vi "Process.vi"(8 "error in":errorcluster, 11 "Qbus in":refnum<class "Qbus.lvclass">) -> (0 "error out":errorcluster)   [LabVIEW 2021, in "AudioGenTCPReaderProcess.lvlib"]
uses:
  AudioGenTCPReaderProcess.lvlib
  <vilib>/addons/Qbus/Qbus.lvclass
  <vilib>/NI/STM/TCP/TCP Read Options.ctl
  shared/logger process/controls/event.ctl
  controls/digital generation settings.ctl
  controls/digital protocol settings.ctl
  <vilib>/PDM Acquisition Toolkit/host/Classes/Session/Controls/Logic Levels.ctl
  <vilib>/PDM Acquisition Toolkit/shared/controls/PCM Data Format Configuration.ctl
  <vilib>/PDM Acquisition Toolkit/shared/controls/Digital Edge.ctl
  <vilib>/PDM Acquisition Toolkit/shared/controls/PCM Bit Endianness.ctl
  <vilib>/PDM Acquisition Toolkit/shared/controls/PCM Data Justification.ctl
  <vilib>/PDM Acquisition Toolkit/shared/controls/clock mode.ctl
  <vilib>/PDM Acquisition Toolkit/shared/controls/PCM Frame Sync Control.ctl
  controls/signal settings.ctl
  controls/signal type.ctl
  shared/controls/digital output level units.ctl
  controls/analog generation settings.ctl
  controls/analog output settings.ctl
  controls/terminal configuration.ctl
  <vilib>/NI/STM/TCP/Read Message (TCP).vi
  <vilib>/NI/STM/TCP/Write Message (TCP).vi
  ManageConnection/AudioGenManageConnectionProcess.lvlib
  <vilib>/NI/STM/NI STM.lvlib
  shared/logger process/EventLoggerProcess.lvlib
  Digital Audio Generation/DigitalAudioGenerationProcess.lvlib
  <vilib>/PDM Acquisition Toolkit/host/Classes/Session/DecoderSession.lvclass
  <vilib>/PDM Acquisition Toolkit/shared/PDM Shared.lvlib
  controls/AudioGenTypeDefs.lvlib
  subVIs/utility/AudioGenUtility.lvlib
  Analog Generation/AnalogGenerationProcess.lvlib
  shared/controls/audio controls.lvlib
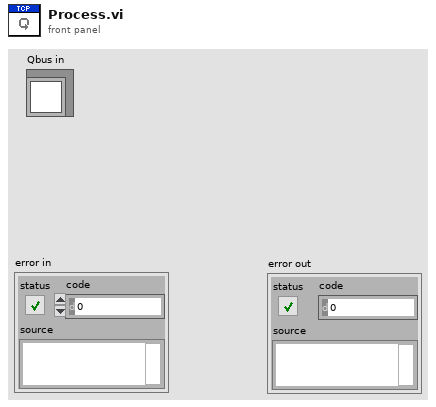
[diagram p1: front panel]
types:
  T1 = typedef "NI STM.lvlib/TCP Read Options.ctl" = cluster{"ignore timeout error":bool, "timeout ms (1000)":i32}
  T2 = typedef "EventLoggerProcess.lvlib/event.ctl" = cluster{"name":string, "description":string}
  T3 = typedef "AudioGenTypeDefs.lvlib/digital generation settings.ctl" = cluster{"data channel list":string, "master clock channel list":string, "digital protocol settings":T4, "signal settings":T12}
  T4 = typedef "AudioGenTypeDefs.lvlib/digital protocol settings.ctl" = cluster{"logic level":T5, "PCM Data Configuration":T6, "bit clock rate":sgl, "master clock rate":sgl, "clock mode":T10, "Frame Sync Clock Control":T11}
  T5 = typedef "PDM Acquisition Class Library.lvlib/DecoderSession.lvclass/Logic Levels.ctl" = enum16{"3.3 V", "1.8 V", "1.2 V"}
  T6 = typedef "PDM Shared.lvlib/PCM Data Format Configuration.ctl" = cluster{"Frame Sync Edge for Channel 0":T7, "Channel Count Per Frame":u8, "Channel Length":u16, "Bit Depth":u8, "Channel 0 Offset":u16, "Endianness":T8, "Data Justification":T9}
  T7 = typedef "PDM Shared.lvlib/Digital Edge.ctl" = enum8{"Rising", "Falling"}
  T8 = typedef "PDM Shared.lvlib/PCM Bit Endianness.ctl" = enum16{"MSB First", "LSB First"}
  T9 = typedef "PDM Shared.lvlib/PCM Data Justification.ctl" = enum16{"Left Justified", "Right Justified"}
  T10 = typedef "PDM Shared.lvlib/clock mode.ctl" = enum16{"divided clock", "DDS"}
  T11 = typedef "PDM Shared.lvlib/PCM Frame Sync Control.ctl" = cluster{"Frame Length":u16, "Frame Sync Pulse Width":u16, "Bit Clock Edge  Sync":T7}
  T12 = typedef "AudioGenTypeDefs.lvlib/signal settings.ctl" = cluster{"signal type":T13, "properties":string, "output level units":T14}
  T13 = typedef "AudioGenTypeDefs.lvlib/signal type.ctl" = enum16{"Sine", "Dual Tone"}
  T14 = typedef "audio controls.lvlib/digital output level units.ctl" = enum32{"% FS", "dBFS", "V"}
  T15 = typedef "AudioGenTypeDefs.lvlib/analog generation settings.ctl" = cluster{"channel list":string, "output settings":T16, "signal settings":T12}
  T16 = typedef "AudioGenTypeDefs.lvlib/analog output settings.ctl" = cluster{"output rate":dbl, "range":dbl, "terminal configuration":T17, "output impedance":dbl, "common mode offset":dbl, "pure tone mode":bool}
  T17 = typedef "AudioGenTypeDefs.lvlib/terminal configuration.ctl" = enum32{"Default", "RSE", "Differential", "Pseudodifferential"}
  T18 = typedef "AudioGenTypeDefs.lvlib/service settings.ctl" = cluster{"port":u32, "enable debug log":bool}
  T19 = typedef "NI STM.lvlib/TCP Connection Info.ctl" = cluster{"connection ID":refnum<k5>, "meta data":T20[]}
  T20 = typedef "NI STM.lvlib/MetaDataElement.ctl" = string
  T21 = typedef "AudioGenTypeDefs.lvlib/generation type and status.ctl" = cluster{"status":T22, "generation type":T23}
  T22 = typedef "AudioGenTypeDefs.lvlib/generation status.ctl" = enum16{"Idle", "Committed", "Active"}
  T23 = typedef "AudioGenTypeDefs.lvlib/generation type.ctl" = enum16{"analog", "digital"}
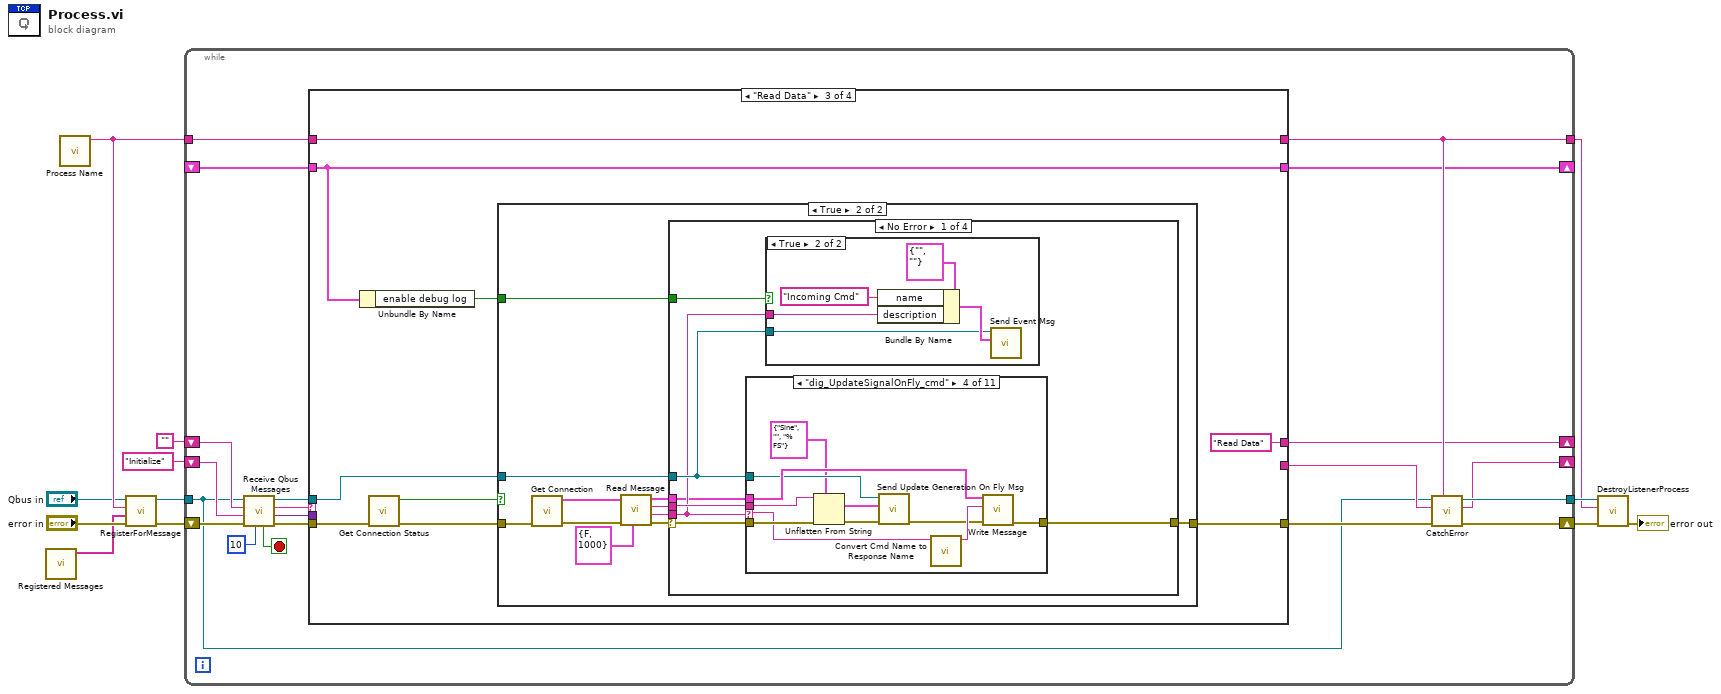
[diagram p0: block diagram]
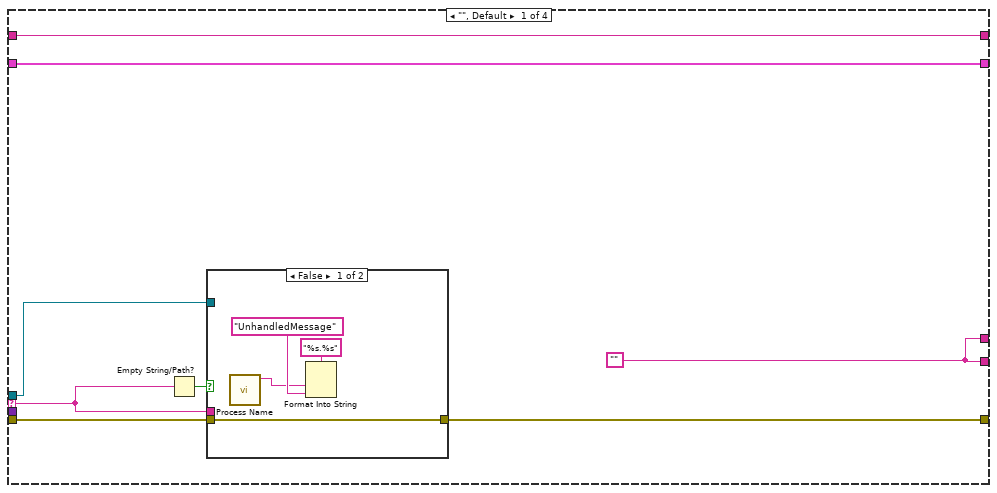
[diagram p2: hidden frame]
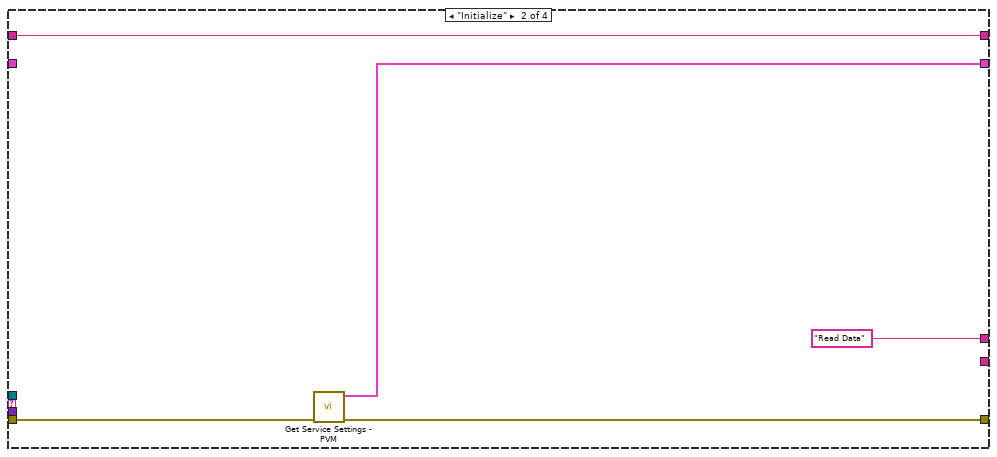
[diagram p4: hidden frame]
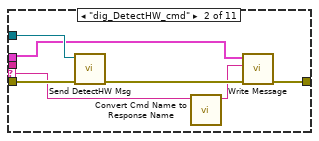
[diagram p8: hidden frame]
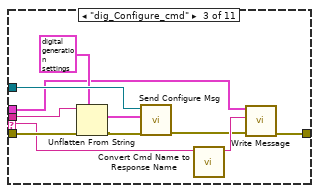
[diagram p9: hidden frame]
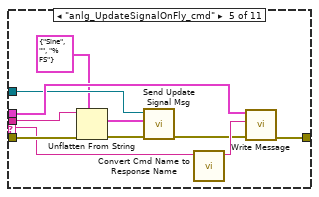
[diagram p10: hidden frame]
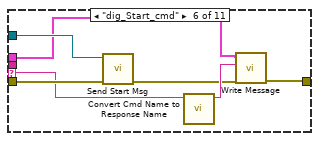
[diagram p11: hidden frame]
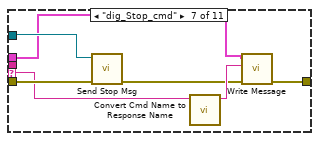
[diagram p12: hidden frame]
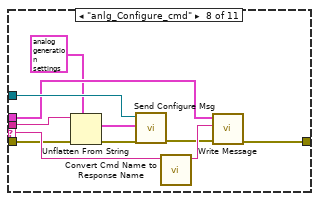
[diagram p13: hidden frame]
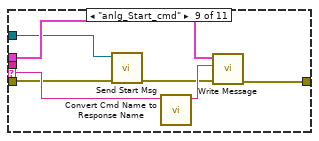
[diagram p14: hidden frame]
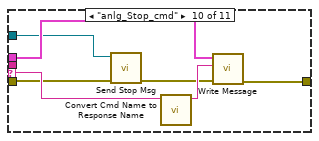
[diagram p15: hidden frame]
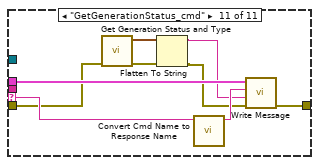
[diagram p16: hidden frame]
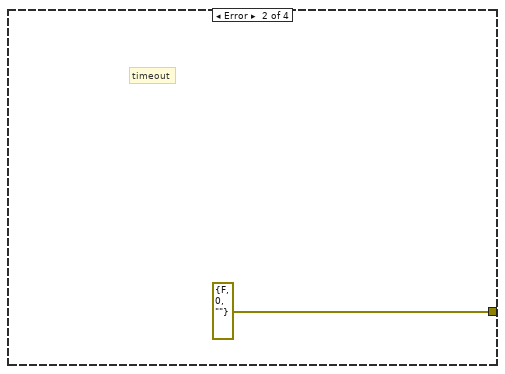
[diagram p17: hidden frame]
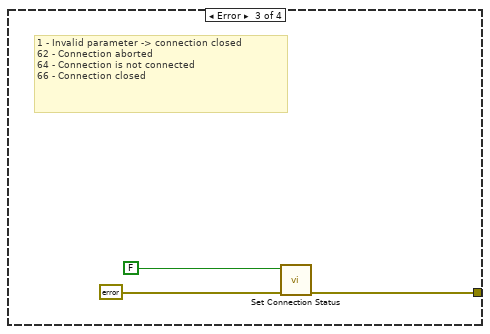
[diagram p18: hidden frame]
diagram:
  n1 = call "Registered Messages.vi"() -> ("registered messages"=w5:string[])  [unwired: 11 in]
  n2 = call "Process Name.vi"() -> ("process name"=w8:string)  [unwired: 11 in]
  n3 = call <vilib>:"RegisterForMessage.vi"("error in (no error)"="error in", "message names"=w5, "process name"=w8, "Qbus in"="Qbus in") -> ("error in (no error)"=w11:errorcluster, "Qbus out"=w12:refnum<class "Qbus.lvclass">)  [unwired: 6 in]
  n4 = while {
    shift-right: [w18] -> _
    shift-left: "" -> [w31]
    tunnel: w12 -> [w16]
    tunnel: w8 -> [w15]
    tunnel: [w25] -> w3
    tunnel: [w20] -> w1
    shift-right: [w24] -> _
    shift-left: "Initialize" -> [w27]
    shift-right: [w26] -> w4
    shift-left: w11 -> [w23]
    shift-right: [w14] -> _
    shift-left: _ -> [w13]
    stop <- w32 stop-if-true
    n5 = call "Receive Qbus Messages.vi"("timeout(ms)"=10 ("milliseconds to wait"), "error in (no error)"=w23, "priority action"=w27, "default action"=w31, "Qbus in"=w16) -> ("error out"=w30:errorcluster, "message value"=w28:variant, "action"=w22:string, "Qbus out"=w29:refnum<class "Qbus.lvclass">, "exit"=w32:bool)  [unwired: 2 in]
    n6 = case shown="\"Read Data\"" w22 {
      selector: w22 -> [w37 _ _ _]
      tunnel: w30 -> [w39 w48 w58 w180]
      tunnel: w29 -> [w35 _ w54 _]
      tunnel: [w38 w47 w53 w180] -> w17
      tunnel: w28 -> [_ _ _ _]
      tunnel: [w40 w50 w59 w179] -> w20
      tunnel: w15 -> [w40 w50 w59 w179]
      tunnel: [w34 _ _ _] -> w19
      tunnel: [w34 "Read Data" "Read Data" _] -> w18
      tunnel: [w33 w46 w52 w178] -> w14
      tunnel: w13 -> [w33 _ w52 w178]
      frame "", Default {
        w34 = ""
        n7 = Empty String/Path?(string/path=w37) -> (empty?=w36:bool)
        n8 = case shown="False" w36 {
          tunnel: [w41 w45] -> w38
          tunnel: w39 -> [w41 w45]
          tunnel: w37 -> [_ _]
          tunnel: w35 -> [_ _]
          frame False {
            n9 = call "Process Name.vi"() -> ("process name"=w42:string)  [unwired: 11 in]
            n10 = Format Into String(format string="%s.%s", w42, "UnhandledMessage" ("ProcessName")) -> ()  [unwired: 2 in, 2 out]
          }
          frame True {
          }
        }
      }
      frame "Initialize" {
        n11 = call "Get Service Settings - PVM.vi"("error in (no error)"=w48) -> ("error out"=w47:errorcluster, "service settings"=w46:T18)  [unwired: 9 in]
      }
      frame "Read Data" {
        n12 = Unbundle By Name(w52) -> ("enable debug log"=w51:bool)
        n13 = call "Get Connection Status.vi"("error in (no error)"=w58) -> ("error out"=w56:errorcluster, "connected"=w57:bool)  [unwired: 9 in]
        n14 = case shown="True" w57 {
          tunnel: w56 -> [w60 w71]
          tunnel: [w60 w65] -> w53
          tunnel: w54 -> [_ w68]
          tunnel: w51 -> [_ w61]
          frame False {
          }
          frame True {
            n15 = call "Get Connection.vi"("error in (no error)"=w71) -> ("error out"=w70:errorcluster, "connection"=w69:T19)  [unwired: 9 in]
            n16 = call-poly <vilib>:"Read Message.vi"("options"=T1 {"ignore timeout error"=FALSE, "timeout ms (1000)"=1000}, "error in"=w70, "connection info in"=w69) -> ("error out"=w63:errorcluster, "name"=w66:T20, "data string"=w67:string, "connection info out"=w62:T19)  [unwired: 3 in, 2 out]
            n17 = case shown="No Error" w63 {
              selector: w63 -> [w77 _ _ w177]
              tunnel: w68 -> [w78 _ _ _]
              tunnel: w67 -> [w76 _ _ _]
              tunnel: w66 -> [w75 _ _ _]
              tunnel: [w73 errorcluster {"status"=FALSE, "code"=0, "source"=""} ("error out") w176 w177] -> w65
              tunnel: w62 -> [w74 _ _ _]
              tunnel: w61 -> [w72 _ _ _]
              frame No Error {
                n18 = case shown="\"dig_UpdateSignalOnFly_cmd\"" w75 {
                  selector: w75 -> [_ w86 w93 w109 w120 w125 w132 w145 w154 w161 w169]
                  tunnel: w77 -> [w84 w91 w101 w113 w124 w131 w137 w143 w151 w159 w166]
                  tunnel: [w84 w88 w92 w108 w119 w127 w134 w147 w155 w162 w170] -> w73
                  tunnel: w78 -> [_ w90 w102 w105 w116 w130 w138 w146 w152 w157 _]
                  tunnel: w76 -> [_ _ w99 w112 w123 _ _ w141 _ _ _]
                  tunnel: w74 -> [_ w87 w94 w110 w121 w126 w133 w144 w153 w160 w171]
                  frame "", Default {
                  }
                  frame "dig_DetectHW_cmd" {
                    n19 = call "Send DetectHW Msg.vi"("error in"=w91, "Qbus in"=w90) -> ("error out"=w89:errorcluster)  [unwired: 8 in, 1 out]
                    n20 = call "Convert Cmd Name to Response Name.vi"("cmd name"=w86) -> ("response name"=w85:string)  [unwired: 10 in]
                    n21 = call-poly <vilib>:"Write Message.vi"("error in"=w89, "name"=w85, "connection info in"=w87) -> ("error out"=w88:errorcluster)  [unwired: 7 in, 1 out]
                  }
                  frame "dig_Configure_cmd" {
                    n22 = Unflatten From String(type=T3 {"data channel list"="", "master clock channel list"="", "digital protocol settings"={"logic level"=enum."3.3 V", "PCM Data Configuration"={"Frame Sync Edge for Channel 0"=enum."Falling", "Channel Count Per Frame"=2, "Channel Length"=32, "Bit Depth"=24, "Channel 0 Offset"=1, "Endianness"=enum."MSB First", "Data Justification"=enum."Left Justified"}, "bit clock rate"=3025000.0, "master clock rate"=3025000.0, "clock mode"=enum."divided clock", "Frame Sync Clock Control"={"Frame Length"=64, "Frame Sync Pulse Width"=32, "Bit Clock Edge  Sync"=enum."Falling"}}, "signal settings"={"signal type"=enum."Sine", "properties"="", "output level units"=enum."% FS"}} ("digital generation"), binary string=w99, error in (no error)=w101) -> (value=w97:T3, error out=w100:errorcluster)  [unwired: 2 in, 1 out]
                    n23 = call "Send Configure Msg.vi"("error in"=w100, "digital generation"=w97, "Qbus in"=w102) -> ("error out"=w95:errorcluster)  [unwired: 7 in, 1 out]
                    n24 = call "Convert Cmd Name to Response Name.vi"("cmd name"=w93) -> ("response name"=w96:string)  [unwired: 10 in]
                    n25 = call-poly <vilib>:"Write Message.vi"("error in"=w95, "name"=w96, "connection info in"=w94) -> ("error out"=w92:errorcluster)  [unwired: 7 in, 1 out]
                  }
                  frame "dig_UpdateSignalOnFly_cmd" {
                    n26 = Unflatten From String(type=T12 {"signal type"=enum."Sine", "properties"="", "output level units"=enum."% FS"} ("signal settings"), binary string=w112, error in (no error)=w113) -> (value=w104:T12, error out=w107:errorcluster)  [unwired: 2 in, 1 out]
                    n27 = call "Send Update Generation On Fly Msg.vi"("error in"=w107, "signal settings"=w104, "Qbus in"=w105) -> ("error out"=w106:errorcluster)  [unwired: 7 in, 1 out]
                    n28 = call "Convert Cmd Name to Response Name.vi"("cmd name"=w109) -> ("response name"=w111:string)  [unwired: 10 in]
                    n29 = call-poly <vilib>:"Write Message.vi"("error in"=w106, "name"=w111, "connection info in"=w110) -> ("error out"=w108:errorcluster)  [unwired: 7 in, 1 out]
                  }
                  frame "anlg_UpdateSignalOnFly_cmd" {
                    n30 = Unflatten From String(type=T12 {"signal type"=enum."Sine", "properties"="", "output level units"=enum."% FS"} ("signal settings"), binary string=w123, error in (no error)=w124) -> (value=w114:T12, error out=w117:errorcluster)  [unwired: 2 in, 1 out]
                    n31 = call "Send Update Signal Msg.vi"("error in"=w117, "signal settings"=w114, "Qbus in"=w116) -> ("error out"=w118:errorcluster)  [unwired: 7 in, 1 out]
                    n32 = call "Convert Cmd Name to Response Name.vi"("cmd name"=w120) -> ("response name"=w122:string)  [unwired: 10 in]
                    n33 = call-poly <vilib>:"Write Message.vi"("error in"=w118, "name"=w122, "connection info in"=w121) -> ("error out"=w119:errorcluster)  [unwired: 7 in, 1 out]
                  }
                  frame "dig_Start_cmd" {
                    n34 = call "Send Start Msg.vi"("error in"=w131, "Qbus in"=w130) -> ("error out"=w128:errorcluster)  [unwired: 8 in, 1 out]
                    n35 = call "Convert Cmd Name to Response Name.vi"("cmd name"=w125) -> ("response name"=w129:string)  [unwired: 10 in]
                    n36 = call-poly <vilib>:"Write Message.vi"("error in"=w128, "name"=w129, "connection info in"=w126) -> ("error out"=w127:errorcluster)  [unwired: 7 in, 1 out]
                  }
                  frame "dig_Stop_cmd" {
                    n37 = call "Send Stop Msg.vi"("error in"=w137, "Qbus in"=w138) -> ("error out"=w135:errorcluster)  [unwired: 8 in, 1 out]
                    n38 = call "Convert Cmd Name to Response Name.vi"("cmd name"=w132) -> ("response name"=w136:string)  [unwired: 10 in]
                    n39 = call-poly <vilib>:"Write Message.vi"("error in"=w135, "name"=w136, "connection info in"=w133) -> ("error out"=w134:errorcluster)  [unwired: 7 in, 1 out]
                  }
                  frame "anlg_Configure_cmd" {
                    n40 = Unflatten From String(type=T15 {"channel list"="", "output settings"={"output rate"=0.0, "range"=0.0, "terminal configuration"=enum."Pseudodifferential", "output impedance"=0.0, "common mode offset"=0.0, "pure tone mode"=FALSE}, "signal settings"={"signal type"=enum."Sine", "properties"="", "output level units"=enum."% FS"}} ("analog generation"), binary string=w141, error in (no error)=w143) -> (value=w139:T15, error out=w142:errorcluster)  [unwired: 2 in, 1 out]
                    n41 = call "Send Configure Msg.vi"("error in"=w142, "analog generation"=w139, "Qbus in"=w146) -> ("error out"=w148:errorcluster)  [unwired: 7 in, 1 out]
                    n42 = call "Convert Cmd Name to Response Name.vi"("cmd name"=w145) -> ("response name"=w149:string)  [unwired: 10 in]
                    n43 = call-poly <vilib>:"Write Message.vi"("error in"=w148, "name"=w149, "connection info in"=w144) -> ("error out"=w147:errorcluster)  [unwired: 7 in, 1 out]
                  }
                  frame "anlg_Start_cmd" {
                    n44 = call "Send Start Msg.vi"("error in"=w151, "Qbus in"=w152) -> ("error out"=w150:errorcluster)  [unwired: 8 in, 1 out]
                    n45 = call "Convert Cmd Name to Response Name.vi"("cmd name"=w154) -> ("response name"=w156:string)  [unwired: 10 in]
                    n46 = call-poly <vilib>:"Write Message.vi"("error in"=w150, "name"=w156, "connection info in"=w153) -> ("error out"=w155:errorcluster)  [unwired: 7 in, 1 out]
                  }
                  frame "anlg_Stop_cmd" {
                    n47 = call "Send Stop Msg.vi"("error in"=w159, "Qbus in"=w157) -> ("error out"=w158:errorcluster)  [unwired: 8 in, 1 out]
                    n48 = call "Convert Cmd Name to Response Name.vi"("cmd name"=w161) -> ("response name"=w163:string)  [unwired: 10 in]
                    n49 = call-poly <vilib>:"Write Message.vi"("error in"=w158, "name"=w163, "connection info in"=w160) -> ("error out"=w162:errorcluster)  [unwired: 7 in, 1 out]
                  }
                  frame "GetGenerationStatus_cmd" {
                    n50 = call "Get Generation Status and Type.vi"("error in (no error)"=w166) -> ("error out"=w165:errorcluster, "type and status"=w164:T21)  [unwired: 9 in]
                    n51 = Flatten To String(anything=w164, error in (no error)=w165) -> (data string=w168:string, error out=w167:errorcluster)  [unwired: 2 in, 1 out]
                    n52 = call "Convert Cmd Name to Response Name.vi"("cmd name"=w169) -> ("response name"=w172:string)  [unwired: 10 in]
                    n53 = call-poly <vilib>:"Write Message.vi"("error in"=w167, "data"=w168, "name"=w172, "connection info in"=w171) -> ("error out"=w170:errorcluster)  [unwired: 6 in, 1 out]
                  }
                }
                n54 = case shown="True" w72 {
                  tunnel: w78 -> [_ w80]
                  tunnel: w75 -> [_ w79]
                  frame False {
                  }
                  frame True {
                    n55 = Bundle By Name(cluster=T2 {"name"="", "description"=""} ("event"), "name"="Incoming Cmd", "description"=w79) -> (w81:T2)
                    n56 = call "Send Event Msg.vi"("event"=w81, "Qbus in"=w80) -> ()  [unwired: 8 in, 2 out]
                  }
                }
              }
              frame Error {
                # "timeout"
              }
              frame Error {
                # "1 - Invalid parameter -> connection closed\n62 - Connection aborted\n64 - Connection is not connected\n66 - Connection closed"
                n57 = call "Set Connection Status.vi"("error in (no error)"=errorcluster {"status"=FALSE, "code"=0, "source"=""}, "connected"=FALSE) -> ("error out"=w176:errorcluster)  [unwired: 9 in]
              }
              frame Default {
              }
            }
          }
        }
      }
      frame "Exit" {
      }
    }
    n58 = call <vilib>:"CatchError.vi"("source"=w20, "error in (no error)"=w17, "next action in"=w19, "Qbus in"=w16) -> ("error out"=w26:errorcluster, "next action out"=w24:string, "Qbus out"=w25:refnum<class "Qbus.lvclass">)  [unwired: 5 in]
  }
  n59 = call <vilib>:"DestroyListenerProcess.vi"("error in (no error)"=w4, "process name"=w1, "Qbus in"=w3) -> ("error in (no error)"=→"error out":errorcluster)  [unwired: 7 in, 1 out]
